vi "Handle New Client.vi"(8 "error in (no error)":errorcluster, 10 "WS Client":refnum<class "WebSocket Client.lvclass">, 11 "WebSocket Handler in":refnum<class "WebSocket Handler.lvclass">) -> (0 "error out":errorcluster, 3 "WebSocket Handler out":refnum<class "WebSocket Handler.lvclass">)   [LabVIEW 2020, in "HTTP Server.lvlib" / "WebSocket Handler.lvclass"]
uses:
  WebSocket Handler.lvclass
  WebSocket Client/WebSocket Client.lvclass
  WebSocket Client/WebSocket Client.lvclass/WebSocket Client.ctl
  lv-http-util/HTTP Utils/Request/Request.lvclass/Request.ctl
  lv-uri/URI/URI/URI.lvclass/URI.ctl
  lv-http-util/HTTP Utils/Request/Get Target URI.vi
  lv-uri/URI/URI/Path String.vi
  WebSocket Manager/WebSocket Manager.lvclass
  WebSocket Handler.lvclass/WebSocket Handler.ctl
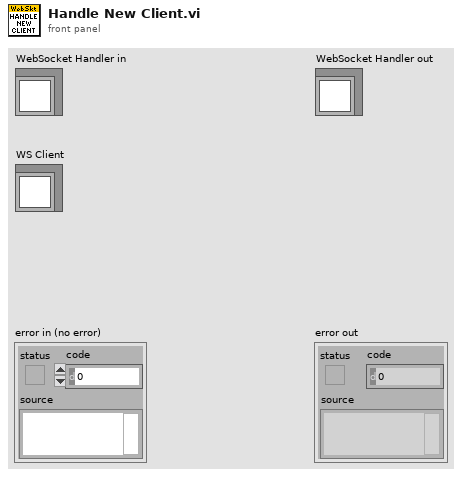
[diagram p1: front panel]
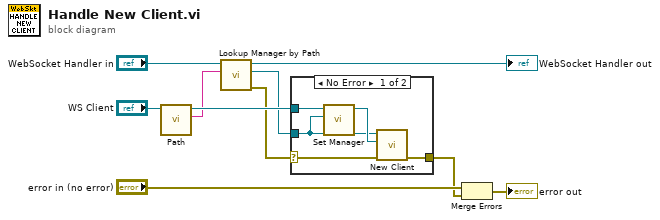
[diagram p0: block diagram]
diagram:
  n1 = call "Path.vi"("WebSocket Client in"="WS Client") -> ("Path"=w3:string, "WebSocket Client out"=w7:refnum<class "WebSocket Client.lvclass">)  [unwired: 9 in]
  n2 = call "Lookup Manager by Path.vi"("Path"=w3, "WebSocket Handler in"="WebSocket Handler in") -> ("error out"=w2:errorcluster, "Manager"=w1:refnum<class "WebSocket Manager.lvclass">, "WebSocket Handler out"=→"WebSocket Handler out":refnum<class "WebSocket Handler.lvclass">)  [unwired: 7 in]
  n3 = case shown="No Error" w2 {
    selector: w2 -> [w11 w16]
    tunnel: w1 -> [w12 _]
    tunnel: w7 -> [w15 _]
    tunnel: [w14 w16] -> w5
    frame No Error {
      n4 = call "Set Manager.vi"("Manager"=w12, "WebSocket Client in"=w15) -> ("WebSocket Client out"=w13:refnum<class "WebSocket Client.lvclass">)  [unwired: 9 in]
      n5 = call "New Client.vi"("error in (no error)"=w11, "WebSocket Client"=w13, "WebSocket Manager in"=w12) -> ("error out"=w14:errorcluster)  [unwired: 8 in]
    }
    frame Error {
    }
  }
  n6 = Merge Errors("error in (no error)", w5) -> (→"error out":errorcluster)
